vi "Device INI path.vi"() -> (3 "appended path":path)   [LabVIEW 2021]
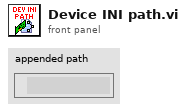
[diagram p1: front panel]
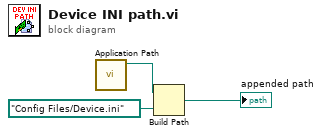
[diagram p0: block diagram]
diagram:
  n1 = call "Application Path.vi"() -> ("appended path"=w3:path)  [unwired: 11 in]
  n2 = Build Path(base path=w3, name or relative path=path "Config Files/Device.ini" ("configuration file path")) -> (appended path=→"appended path":path)
